vi "Set Build Specification Version.vi"(6 "Build Specification Version":T1, 8 "error in":errorcluster, 9 "Build Specification":string, 10 "Project File":path, 11 "Project Manager in":refnum<class "Project Manager.lvclass">) -> (0 "error out":errorcluster, 3 "Project Manager out":refnum<class "Project Manager.lvclass">)   [LabVIEW 2026, in "Project Manager.lvclass"]
doc: "Set version of build specification (in target My Computer)."
uses:
  Project Manager.lvclass
  <vilib>/AppBuilder/AB_API_Simple/Build Specification Version.ctl
  <vilib>/AppBuilder/AB_API_Simple/Set Build Specification Version (path).vi
  <vilib>/AppBuilder/AB_API_Simple/NI_App_Builder_API.lvlib
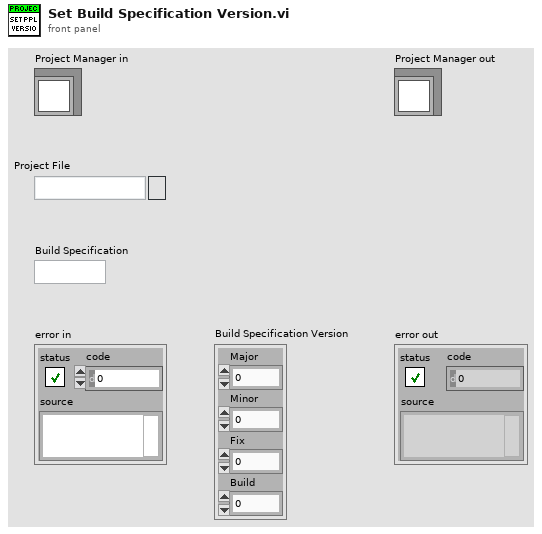
[diagram p1: front panel]
types:
  T1 = typedef "NI_App_Builder_API.lvlib/Build Specification Version.ctl" = cluster{"Major":u16, "Minor":u16, "Fix":u16, "Build":u16}
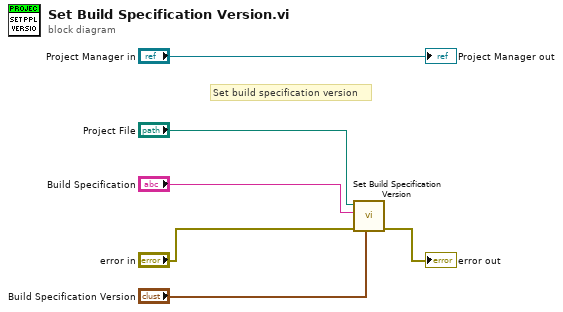
[diagram p0: block diagram]
diagram:
  # "Set build specification version"
  n1 = call-poly <vilib>:"Set Build Specification Version.vi"("Build Specification Version"="Build Specification Version", "error in (no error)"="error in", "Name of build specification"="Build Specification", "Path to project"="Project File") -> ("error out"=→"error out":errorcluster)  [unwired: 7 in]
  "Project Manager out" <- "Project Manager in"
